vi "Json to object.vi"(8 "error in":errorcluster, 10 "json":string) -> (0 "error out":errorcluster, 3 "json class out":refnum<class "json class.lvclass">)   [LabVIEW 2021, in "Config Library.lvlib" / "json class.lvclass"]
uses:
  json class.lvclass
  json class.lvclass/json class.ctl
  <vilib>/addons/JSON API/JSON Value/Set from JSON string.vi
  <vilib>/addons/JSON API/JSON Value/JSON Value.lvclass
  <vilib>/addons/JSON API/Get Polymorphic/JSON GetSet.lvlib
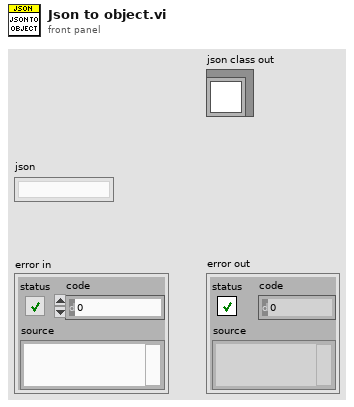
[diagram p1: front panel]
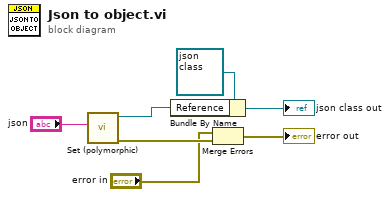
[diagram p0: block diagram]
diagram:
  n1 = call-poly <vilib>:"Set (polymorphic).vi"("JSON stream"="json") -> ("error out"=w7:errorcluster, "JSON Value out"=w5:refnum<class "JSON Value.lvclass">)  [unwired: 8 in, 1 out]
  n2 = Bundle By Name(cluster=refnum<class "json class.lvclass"> refnum ("json class in"), "Reference"=w5) -> (→"json class out":refnum<class "json class.lvclass">)
  n3 = Merge Errors("error in", w7) -> (→"error out":errorcluster)
